vi "RDC-Lin-Calc_Impedance.vi"(10 "Reflection Tip":cdb[](array[numeric])) -> (1 "Admittance":cdb[](array[numeric]), 2 "Impedance":cdb[](array[numeric]))   [LabVIEW 2020, in "RDC-Reflection_Data_Computation.lvlib"]
doc: "Computes the impedance and admittance arrays from a tip reflection array."
uses:
  RDC-Reflection_Data_Computation.lvlib
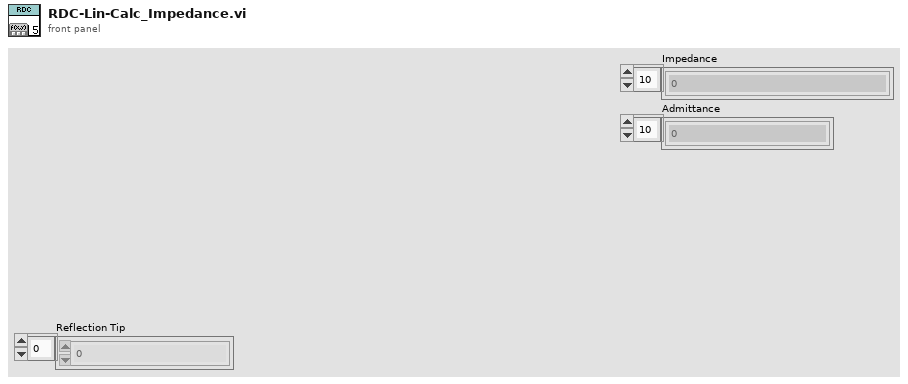
[diagram p1: front panel]
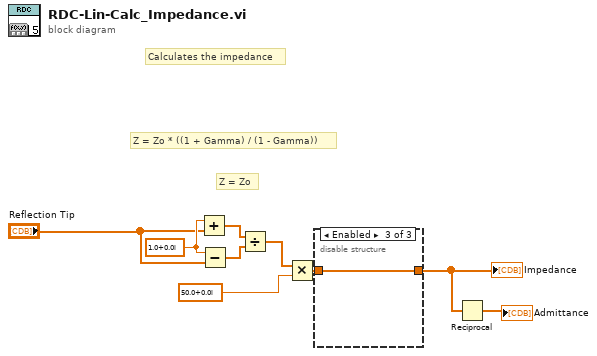
[diagram p0: block diagram]
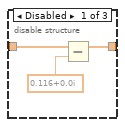
[diagram p2: hidden frame]
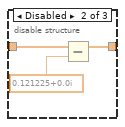
[diagram p3: hidden frame]
diagram:
  w6 = cdb 1.0+0.0i ("x")
  # "Calculates the impedance"
  # "Z = Zo"
  # "Z = Zo * ((1 + Gamma) / (1 - Gamma))"
  n1 = Add(x=w6, y="Reflection Tip") -> (x+y=w7:cdb[])
  n2 = Subtract(x=w6, y="Reflection Tip") -> (x-y=w8:cdb[])
  n3 = Divide(x=w7, y=w8) -> (x/y=w9:cdb[])
  n4 = Multiply(x=w9, y=cdb 50.0+0.0i) -> (x*y=w2:cdb[])
  n5 = disable-structure shown="Enabled" {
    disable-tunnel: w2 -> [w12 w15 w16]
    disable-tunnel: [w11 w14 w16] -> w1
    frame Disabled {
      n6 = Subtract(x=w12, y=cdb 0.116+0.0i ("x")) -> (x-y=w11:cdb[])
    }
    frame Disabled {
      n7 = Subtract(x=w15, y=cdb 0.121225+0.0i ("x")) -> (x-y=w14:cdb[])
    }
    frame Enabled {
    }
  }
  "Impedance" <- w1
  n8 = Reciprocal(x=w1) -> (1/x=→"Admittance":cdb[])
